vi "Create Argument_String.vi"(10 "argument data":string, 11 "argument name":string) -> (3 "argument out":string)   [LabVIEW 2019, in "Error Generation.lvlib"]
doc: "Create an argument string in the format\n\n< b > argument name< /b >\nargument data\n\nIf argument name is empty argument string is empty.\nEmpty argument data are allowed.\n- - -\nCopyright (c) 2023, Merecs Engineering GmbH"
uses:
  Error Generation.lvlib
panel:
  # "Connector Pane"
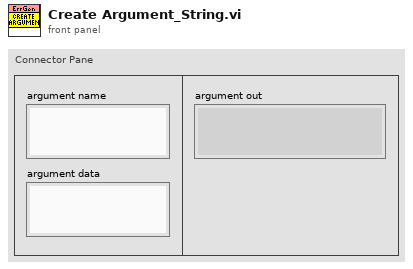
[diagram p1: front panel]
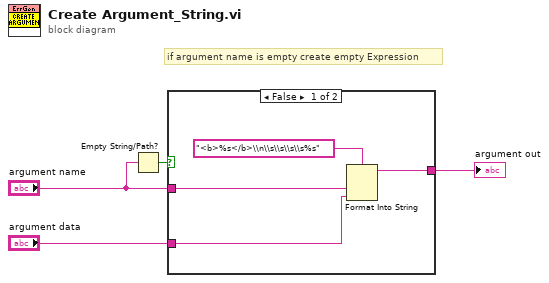
[diagram p0: block diagram]
diagram:
  # "if argument name is empty create empty Expression"
  n1 = Empty String/Path?(string/path="argument name") -> (empty?=w2:bool)
  n2 = case shown="False" w2 {
    tunnel: "argument data" -> [w7 _]
    tunnel: "argument name" -> [w6 w9]
    tunnel: [w5 w9] -> w3
    frame False {
      n3 = Format Into String(format string="<b>%s</b>\\n\\s\\s\\s\\s%s", w6, w7) -> (resulting string=w5:string)  [unwired: 2 in, 1 out]
    }
    frame True {
    }
  }
  "argument out" <- w3
